vi "Fire_waveform.vi"(0 "Camera_trigger_on":bool=TRUE, 1 "gate_start_ms":dbl=230.0, 5 "gate_len_ms":dbl=20.0, 6 "camera_pulse_ms":dbl=50.0, 7 "camera_delay":dbl=50.0, 8 "valve_pulse_ms":dbl=50.0, 9 "valve_delay":dbl=150.0, 10 "rate":dbl=1000.0, 11 "pulse_length_ms":dbl=500.0) -> (2 "N":i32, 3 "waveform":dbl[][](array[numeric]), 4 "Gate":u32[](array[numeric]))   [LabVIEW 2025]
panel:
  out "Waveform Graph":dbl[][](graph)
  in  "amplitude":dbl=4.9
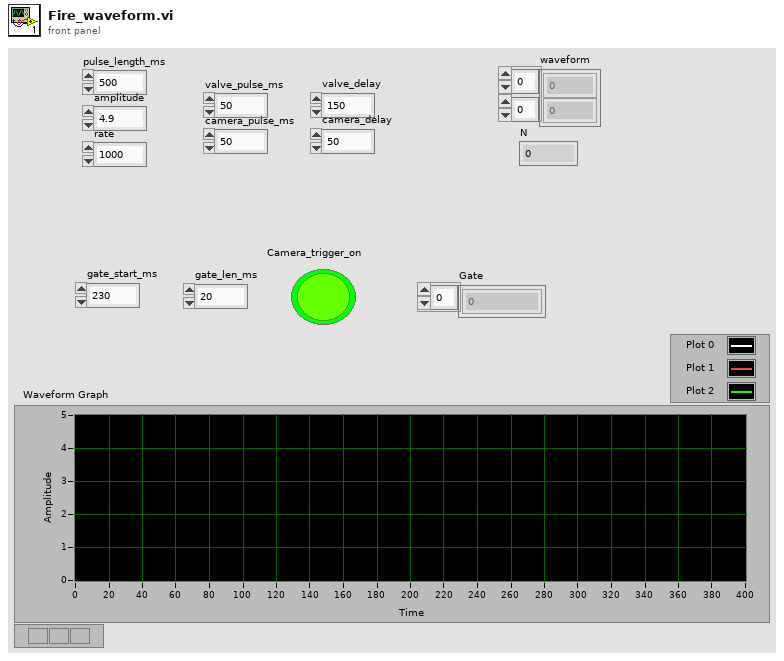
[diagram p1: front panel]
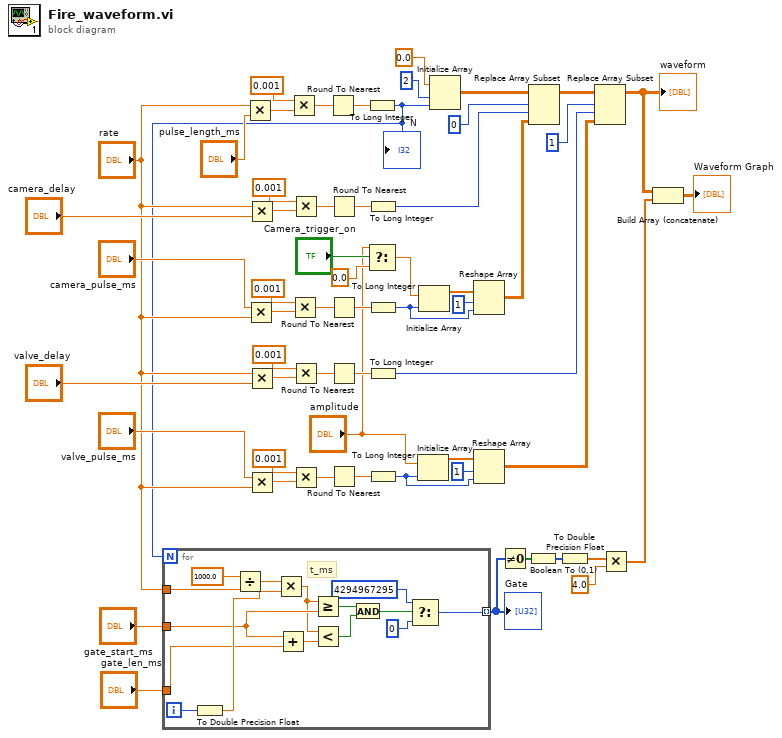
[diagram p0: block diagram]
diagram:
  n1 = Multiply(x="rate", y="pulse_length_ms") -> (x*y=w56:dbl)
  n2 = Multiply(x="camera_pulse_ms", y="rate") -> (x*y=w50:dbl)
  n3 = Multiply(x="rate", y="camera_delay") -> (x*y=w48:dbl)
  n4 = Multiply(x="rate", y="valve_delay") -> (x*y=w44:dbl)
  n5 = Multiply(x="valve_pulse_ms", y="rate") -> (x*y=w42:dbl)
  n6 = Multiply(x=0.001, y=w56) -> (x*y=w54:dbl)
  n7 = Multiply(x=0.001, y=w50) -> (x*y=w34:dbl)
  n8 = Multiply(x=0.001, y=w48) -> (x*y=w37:dbl)
  n9 = Multiply(x=0.001, y=w44) -> (x*y=w32:dbl)
  n10 = Multiply(x=0.001, y=w42) -> (x*y=w30:dbl)
  n11 = Round To Nearest(number=w54) -> (nearest integer value=w53:dbl)
  n12 = Round To Nearest(number=w37) -> (nearest integer value=w38:dbl)
  n13 = Round To Nearest(number=w34) -> (nearest integer value=w35:dbl)
  n14 = Round To Nearest(number=w32) -> (nearest integer value=w33:dbl)
  n15 = Round To Nearest(number=w30) -> (nearest integer value=w31:dbl)
  n16 = To Long Integer(number=w53) -> (32bit integer=w12:i32)
  "N" <- w12
  n17 = for {
    N: w12 -> [_]
    tunnel: "rate" -> [w70]
    tunnel: "gate_start_ms" -> [w66]
    tunnel: "gate_len_ms" -> [w65]
    tunnel: [w58] -> w8 mode=indexing
    i -> [w72]
    # "t_ms"
    n18 = To Double Precision Float(number=w72) -> (double precision float=w68:dbl)
    n19 = Divide(x=1000.0, y=w70) -> (x/y=w69:dbl)
    n20 = Multiply(x=w69, y=w68) -> (x*y=w64:dbl)
    n21 = Add(x=w66, y=w65) -> (x+y=w63:dbl)
    n22 = Greater Or Equal?(x=w64, y=w66) -> (x >= y?=w67:bool)
    n23 = Less?(x=w64, y=w63) -> (x < y?=w62:bool)
    n24 = And(x=w67, y=w62) -> (x .and. y?=w61:bool)
    n25 = Select(t=u32 4294967295, s=w61, f=u32 0) -> (s? t:f=w58:u32)
  }
  "Gate" <- w8
  n26 = Select(t="amplitude", s="Camera_trigger_on", f=0.0) -> (s? t:f=w10:dbl)
  n27 = To Long Integer(number=w38) -> (32bit integer=w36:i32)
  n28 = To Long Integer(number=w35) -> (32bit integer=w27:i32)
  n29 = To Long Integer(number=w33) -> (32bit integer=w25:i32)
  n30 = To Long Integer(number=w31) -> (32bit integer=w24:i32)
  n31 = Initialize Array("amplitude", w24) -> (w23:dbl[])
  n32 = Initialize Array(w10, w27) -> (w29:dbl[])
  n33 = Initialize Array(0.0, 2 ("dimension size"), w12) -> (w46:dbl[][])
  n34 = Reshape Array(w29, 1 ("dimension size"), w27) -> (w26:dbl[][])
  n35 = Reshape Array(w23, 1 ("dimension size"), w24) -> (w21:dbl[][])
  n36 = Not Equal To 0?(x=w8) -> (x != 0?=w7:bool[])
  n37 = Boolean To (0,1)(Boolean=w7) -> (0, 1=w6:i16[])
  n38 = Replace Array Subset(array=w46, new element=w26, index (row)=0, index (col)=w36) -> (w40:dbl[][])
  n39 = To Double Precision Float(number=w6) -> (double precision float=w4:dbl[])
  n40 = Replace Array Subset(array=w40, new element=w21, index (row)=1, index (col)=w25) -> (w3:dbl[][])
  "waveform" <- w3
  n41 = Multiply(x=w4, y=4.0) -> (x*y=w2:dbl[])
  n42 = Build Array (concatenate)(w3, w2) -> (→"Waveform Graph":dbl[][])
